vi "Watchdog Add Trigger Action.vi"(4 "error in (no error)":errorcluster, 5 "trigger protocol":T1(ring), 6 "trigger ID":u32=4, 7 "watchdogID in":u64 format="%.0x") -> (0 "error out":errorcluster, 3 "watchdogID out":u64 format="%.0x")   [LabVIEW 2025]
doc: "<p>Configures the <a href=\"nihelplauncher://docs/csh?context=lvrt_lvrtconcepts_rt_watchdog\">watchdog object</a> to assert a PXI trigger line when the watchdog timer expires. Use this VI in the configuration stage of the application, prior to the Watchdog Enable VI.</p>"
uses:
  niwd4c.dll
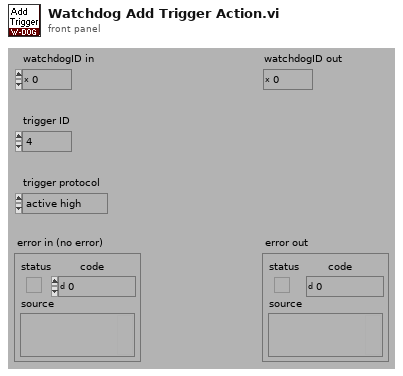
[diagram p1: front panel]
types:
  T1 = enum16{"active high", "active low", "open collector"}
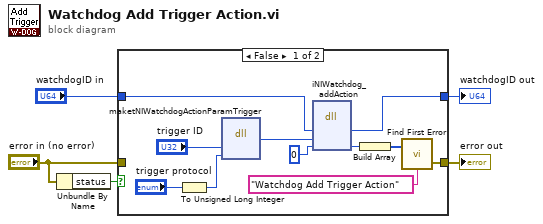
[diagram p0: block diagram]
diagram:
  n1 = Unbundle By Name("error in (no error)") -> ("status"=w5:bool)
  n2 = case shown="False" w5 {
    tunnel: [w11 w17] -> w2
    tunnel: [w15 w18] -> w1
    tunnel: "error in (no error)" -> [_ w18]
    tunnel: "watchdogID in" -> [w9 w17]
    frame False {
      n3 = To Unsigned Long Integer(number="trigger protocol") -> (unsigned 32bit integer=w6:u32)
      n4 = dll-call lib="niwd4c.*" fn="maketNIWatchdogActionParamTrigger" label="Action Trigger"("identifier"="trigger ID", "protocol"=w6) -> ("return type"=w13:u64)  [unwired: 5 in, 2 out]
      n5 = dll-call lib="niwd4c.*" fn="iNIWatchdog_addAction" label="Add Action"("wd"=w9, "parameter"=w13, "status"=0) -> ("wd"=w11:u64, "status"=w12:i32)  [unwired: 5 in, 2 out]
      n6 = Build Array(w12) -> (w16:i32[])
      n7 = call <vilib>:"Find First Error.vi"("source messages"="Watchdog Add Trigger Action", "error codes"=w16) -> ("error out"=w15:errorcluster)  [unwired: 2 in, 1 out]
    }
    frame True {
    }
  }
  "error out" <- w1
  "watchdogID out" <- w2
